vi "FiSpec Data processing_v2_LV2014.vi"(10 "Onboard peak detection":bool, 11 "Data string (without \"Ende\")":string) -> (0 "Reference Compensation: slope":dbl format="%.6f", 1 "Amplitude":u16[](array[numeric]), 2 "Peak amplitudes":dbl[](array[numeric]), 3 "Peak wavelengths":dbl[](array[numeric]), 4 "Reference Compensation: Offset":dbl, 5 "System Temperature":dbl)   [LabVIEW 2017]
panel:
  in  "Firmware>=8.6":bool
  out "Spectrum":u16[](graph)
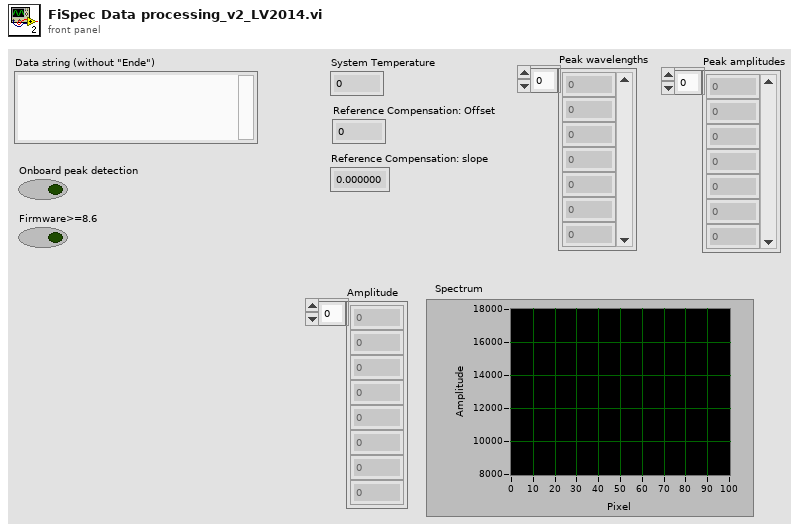
[diagram p1: front panel]
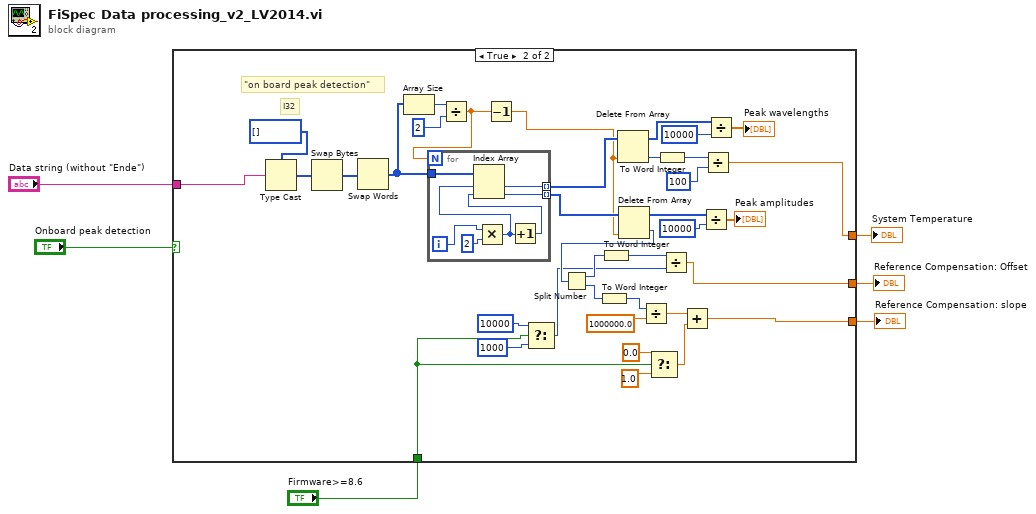
[diagram p0: block diagram]
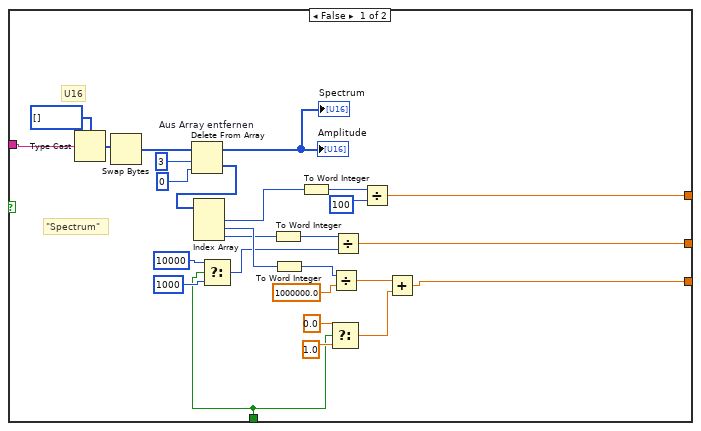
[diagram p2: hidden frame]
diagram:
  n1 = case shown="True" "Onboard peak detection" {
    tunnel: [w21 w47] -> w6
    tunnel: [w20 w46] -> w5
    tunnel: [w8 w35] -> w4
    tunnel: "Data string (without \"Ende\")" -> [w19 w49]
    tunnel: "Firmware>=8.6" -> [w7 w34]
    frame False {
      # "\"Spectrum\""
      # "U16"
      n2 = Type Cast(type=u16[] [] ("Angehängtes Array"), x=w19) -> (*(type *) &x=w17:u16[])
      n3 = Swap Bytes(anything=w17) -> (byte swapped=w16:u16[])
      n4 = Delete From Array "Aus Array entfernen"(array=w16, length=3 ("Länge"), index=0 ("Index")) -> (deleted portion=w29:u16[], array with subset deleted=→"Amplitude" →"Spectrum":u16[])
      n5 = Index Array(array=w29) -> (element #1=w24:u16, element #2=w26:u16, element #3=w25:u16)  [unwired: 3 in]
      n6 = Select(t=i16 10000 ("y"), s=w7, f=i16 1000 ("y")) -> (s? t:f=w13:i16)
      n7 = To Word Integer(number=w25) -> (16bit integer=w27:i16)
      n8 = To Word Integer(number=w26) -> (16bit integer=w28:i16)
      n9 = To Word Integer(number=w24) -> (16bit integer=w23:i16)
      n10 = Select(t=0.0 ("y"), s=w7, f=1.0 ("y")) -> (s? t:f=w9:dbl)
      n11 = Divide(x=w28, y=1000000.0) -> (x/y=w10:dbl)
      n12 = Divide(x=w27, y=w13) -> (x/y=w20:dbl)
      n13 = Divide(x=w23, y=100) -> (x/y=w21:dbl)
      n14 = Add(x=w10, y=w9) -> (x+y=w8:dbl)
    }
    frame True {
      # "I32"
      # "\"on board peak detection\""
      n15 = Type Cast(type=i32[] [] ("Angehängtes Array"), x=w49) -> (*(type *) &x=w44:i32[])
      n16 = Swap Bytes(anything=w44) -> (byte swapped=w45:i32[])
      n17 = Swap Words(1:w45) -> (0:w43:i32[])
      n18 = Array Size(array=w43) -> (size(s)=w69:i32)
      n19 = Divide(x=w69, y=2) -> (x/y=w68:dbl)
      n20 = for {
        N: w68 -> [_]
        tunnel: w43 -> [w77]
        tunnel: [w72] -> w67 mode=indexing
        tunnel: [w71] -> w66 mode=indexing
        i -> [w76]
        n21 = Multiply(x=w76, y=2) -> (x*y=w74:i32)
        n22 = Increment(x=w74) -> (x+1=w73:i32)
        n23 = Index Array(array=w77, index #1=w74, index #2=w73) -> (element #1=w72:i32, element #2=w71:i32)
      }
      n24 = Decrement(x=w68) -> (x-1=w65:dbl)
      n25 = Select(t=i16 10000 ("y"), s=w34, f=i16 1000 ("y")) -> (s? t:f=w40:i16)
      n26 = Delete From Array(array=w67, index=w65) -> (deleted portion=w62:i32, array with subset deleted=w64:i32[])  [unwired: 1 in]
      n27 = Delete From Array(array=w66, index=w65) -> (deleted portion=w56:i32, array with subset deleted=w63:i32[])  [unwired: 1 in]
      n28 = Split Number(x=w56) -> (hi(x)=w59:u16, lo(x)=w60:u16)
      n29 = To Word Integer(number=w60) -> (16bit integer=w57:i16)
      n30 = To Word Integer(number=w59) -> (16bit integer=w58:i16)
      n31 = Divide(x=w57, y=1000000.0) -> (x/y=w37:dbl)
      n32 = Select(t=0.0 ("y"), s=w34, f=1.0 ("y")) -> (s? t:f=w36:dbl)
      n33 = To Word Integer(number=w62) -> (16bit integer=w61:i16)
      n34 = Divide(x=w58, y=w40) -> (x/y=w46:dbl)
      n35 = Add(x=w37, y=w36) -> (x+y=w35:dbl)
      n36 = Divide(x=w63, y=10000) -> (x/y=→"Peak amplitudes":dbl[])
      n37 = Divide(x=w61, y=u16 100) -> (x/y=w47:dbl)
      n38 = Divide(x=w64, y=10000) -> (x/y=→"Peak wavelengths":dbl[])
    }
  }
  "System Temperature" <- w6
  "Reference Compensation: Offset" <- w5
  "Reference Compensation: slope" <- w4
